vi "Flatten Buffer Configuration.vi"(11 "Buffer Configuration":T1) -> (3 "Flattened Configuration":u8[](array[numeric]) format="%.0x")   [LabVIEW 2021, in "CIF_CIPC_Chn.lvclass"]
uses:
  CIF_CIPC_Chn.lvclass
  Typedef/Buffer Configuration Data.ctl
  <vilib>/CIF Foundation/CIF CIPC/TypeDefs/Backpressure References.ctl
  <vilib>/CIF Foundation/CIF CIPC/TypeDefs/Backpressure Names.ctl
  CIF_CIPC_Chn.lvclass/CIF_CIPC_Chn.ctl
  <vilib>/CIF Foundation/CIF Utilities/DataTypes/DataTypes_CIF_U.lvlib
  <vilib>/CIF Foundation/CIF CIPC/CIF_NI_CIPC.lvlib
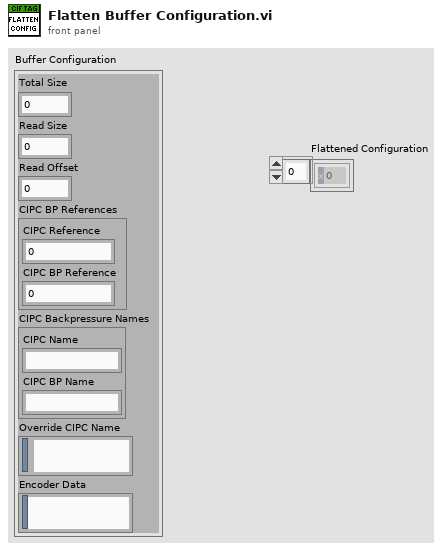
[diagram p1: front panel]
types:
  T1 = typedef "CIF_CIPC_Chn.lvclass/Buffer Configuration Data.ctl" = cluster{"Total Size":u32, "Read Size":u32, "Read Offset":u32, "CIPC BP References":T2, "CIPC Backpressure Names":T3, "Override CIPC Name":string, "Encoder Data":string}
  T2 = typedef "CIF_NI_CIPC.lvlib/Backpressure References.ctl" = cluster{"CIPC Reference":u64, "CIPC BP Reference":u64}
  T3 = typedef "CIF_NI_CIPC.lvlib/Backpressure Names.ctl" = cluster{"CIPC Name":string, "CIPC BP Name":string}
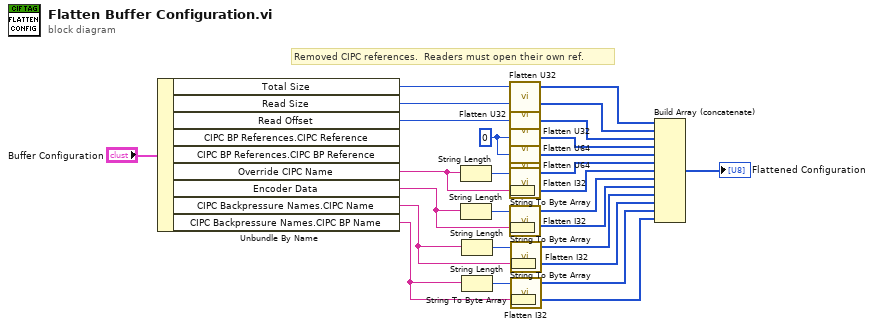
[diagram p0: block diagram]
diagram:
  w1 = u64 0 ("U64")
  # "Removed CIPC references.  Readers must open their own ref."
  n1 = Unbundle By Name("Buffer Configuration") -> ("Total Size"=w26:u32, "Read Size"=w24:u32, "Read Offset"=w25:u32, "Override CIPC Name"=w17:string, "Encoder Data"=w14:string, "CIPC Backpressure Names.CIPC Name"=w9:string, "CIPC Backpressure Names.CIPC BP Name"=w8:string)  [unwired: 2 out]
  n2 = String Length(string=w17) -> (length=w19:i32)
  n3 = String Length(string=w14) -> (length=w15:i32)
  n4 = String Length(string=w9) -> (length=w6:i32)
  n5 = String Length(string=w8) -> (length=w7:i32)
  n6 = String To Byte Array(string=w17) -> (unsigned byte array=w16:u8[])
  n7 = String To Byte Array(string=w14) -> (unsigned byte array=w12:u8[])
  n8 = String To Byte Array(string=w9) -> (unsigned byte array=w4:u8[])
  n9 = String To Byte Array(string=w8) -> (unsigned byte array=w2:u8[])
  n10 = call <vilib>:"Flatten U32.vi"("U32"=w26) -> ("Flat Data"=w23:u8[])  [unwired: 4 in]
  n11 = call <vilib>:"Flatten U32.vi"("U32"=w24) -> ("Flat Data"=w22:u8[])  [unwired: 4 in]
  n12 = call <vilib>:"Flatten U32.vi"("U32"=w25) -> ("Flat Data"=w21:u8[])  [unwired: 4 in]
  n13 = call <vilib>:"Flatten U64.vi"("U64"=w1) -> ("Flat Data"=w10:u8[])  [unwired: 4 in]
  n14 = call <vilib>:"Flatten U64.vi"("U64"=w1) -> ("Flat Data"=w11:u8[])  [unwired: 4 in]
  n15 = call <vilib>:"Flatten I32.vi"("I32"=w19) -> ("Flat Data"=w18:u8[])  [unwired: 4 in]
  n16 = call <vilib>:"Flatten I32.vi"("I32"=w15) -> ("Flat Data"=w13:u8[])  [unwired: 4 in]
  n17 = call <vilib>:"Flatten I32.vi"("I32"=w6) -> ("Flat Data"=w5:u8[])  [unwired: 4 in]
  n18 = call <vilib>:"Flatten I32.vi"("I32"=w7) -> ("Flat Data"=w3:u8[])  [unwired: 4 in]
  n19 = Build Array (concatenate)(w23, w22, w21, w10, w11, w18, w16, w13, w12, w5, w4, w3, w2) -> (→"Flattened Configuration":u8[])
